vi "subscribe.vi"(8 "error in":errorcluster, 9 "Python env version":string="3.12", 10 "Path to client.py":path, 11 "Python env directory":path) -> (0 "error out":errorcluster)   [LabVIEW 2023]
uses:
  <vilib>/Python/Open Venv Python Session.vi
panel:
  in  "Process Stop Button":bool
  out "published value\n(-1 on timeout)":i32
  in  "Service name (Python or LabVIEW)":string="Python"
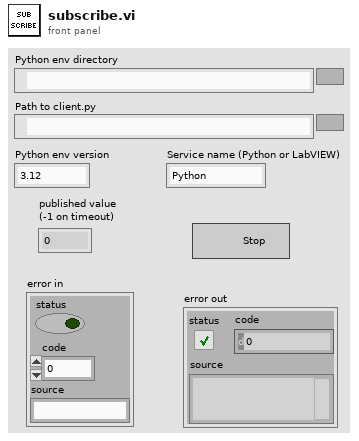
[diagram p1: front panel]
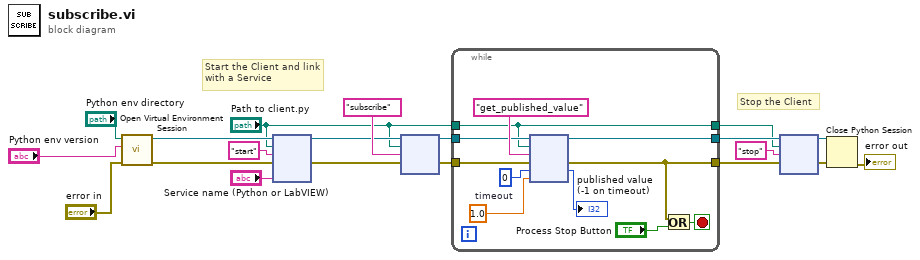
[diagram p0: block diagram]
diagram:
  # "Stop the Client"
  # "Start the Client and link with a Service"
  n1 = call-poly <vilib>:"Open Virtual Environment Session.vi"("error in (no error)"="error in", "Python version"="Python env version", "Env path"="Python env directory") -> ("error out"=w17:errorcluster, "session out"=w18:refnum<k35>)  [unwired: 7 in]
  n2 = node(w18, "Path to client.py", "start" ("function name"), w17, "Service name (Python or LabVIEW)") -> (w7:refnum<k35>, w8:errorcluster)  [unwired: 3 in, 2 out]
  n3 = node(w7, "Path to client.py", "subscribe" ("function name"), w8) -> (w5:refnum<k35>, w6:errorcluster)  [unwired: 2 in, 2 out]
  n4 = while {
    tunnel: w6 -> [w30]
    tunnel: w5 -> [w29]
    tunnel: "Path to client.py" -> [w27]
    tunnel: [w28] -> w3
    tunnel: [w27] -> w2
    tunnel: [w24] -> w1
    stop <- w26 stop-if-true
    w23 = 1.0  # timeout
    n5 = node(w29, w27, "get_published_value" ("function name"), w30, 0, w23) -> (w28:refnum<k35>, w24:errorcluster, →"published value\n(-1 on timeout)":i32)  [unwired: 1 in, 2 out]
    n6 = Or(x=w24, y="Process Stop Button") -> (x .or. y?=w26:bool)
  }
  n7 = node(w3, w2, "stop" ("function name"), w1) -> (w14:refnum<k35>, w11:errorcluster)  [unwired: 2 in, 2 out]
  n8 = Close Python Session(session in=w14, error in=w11) -> (11:→"error out":errorcluster)
